vi "PicoScope3000aExampleRapidBlockBulkOverlapped.vi"() -> ()   [LabVIEW 2010]
uses:
  shared/PicoBuffers.ctl
  <vilib>/Waveform/DWDTOps.llb/DWDT Analog to Digital.vi
  shared/Segment Range.ctl
  shared/Buffer and Transfer Settings.ctl
  shared/Acquisition Settings.ctl
  shared/nSegments.ctl
  PicoScope3000aLib/PicoScope3000aDigitalChannelSettings.ctl
  PicoScope3000aLib/PicoScope3000aAnalogChannelSettings.ctl
panel:
  in  "Trigger Settings":T1={"Trigger Enabled"=FALSE, "Trigger Source"=enum."Channel A", "Trigger Threshold (volts)"=0.0, "Trigger Direction"=2, "Trigger Delay (samples)"=0, "Auto Trigger Time (ms)"=1000} {"Trigger Direction" items=["Above", "Below", "Rising", "Falling", "Rising or Falling"]}
  in  "Channel A Settings":T2={"Enabled"=TRUE, "Coupling"=1, "Range"=6, "Analogue Offset"=0.0, "Bandwidth Limit"=0} {"Bandwidth Limit" items=["Full", "20MHz"]; "Range" items=["10 mV", "20 mV", "50 mV", "100 mV", "200 mV", "500 mV", "1 V", "2 V", "5 V", "10 V", "20 V", "50 V ", "100 V"]; "Coupling" items=["AC", "DC"]}
  out "overflow":i16[](array[numeric]) format="%06b"
  in  "Port 0 Settings":T3={"Enabled"=FALSE, "Logic Level"=9830} {"Logic Level" items=["1.5V TTL"=9830, "2.5V CMOS"=16383]}
  out "USB 3.0 device on non-USB 3.0 Port":bool
  out "USB Powered":bool=TRUE
  out "Device Info":T4={"Driver Version"="2.1.104.3324", "USB Version"="2.0", "Hardware"="1", "Variant"="5244A", "Batch and Serial"="CQ178/007", "Cal Date"="11Jun13", "Kernel Version"="1.0", "Digital HW Version"="1", "Analogue HW Version"="1", "MSO"=FALSE, "Number of channels"=2}
  in  "Stop Display":bool
  out "Capture Complete":bool
  in  "Run":bool
  in  "Display Buffer Index":i32
  in  "Segment Range":T5={"fromSegmentIndex"=0, "toSegmentIndex"=9} {"toSegmentIndex" format="%.4p"; "fromSegmentIndex" format="%.4p"}
  in  "nSegments":T6=10 format="%.4p"
  out "error out":errorcluster
  in  "Data file":path=path "PicoScope3000aExampleRapidBlock ChA Data"
  in  "Buffer and Transfer Settings":T7={"startIndex"=0, "Samples"=5000000, "Down Sample Ratio"=1, "Down-Sample Mode"=0} {"Down-Sample Mode" items=["RAW none"=2147483648, "None"=0, "Aggregate"=1, "Decimate"=2, "Average"=4]; "Down Sample Ratio" step=1; "Samples" format="%_6p"}
  in  "Acquisition Settings":T8={"preTriggerSamples"=0, "postTriggerSamples"=5000000, "timebase"=5} {"postTriggerSamples" format="%_6p"; "preTriggerSamples" format="%_6p"}
  out "Properties Panel":T9={"Sample Frequency"=41666668.0, "Sample Rate"=2.4000000209412065e-08, "Max Samples Available"=26843008, "Number of Samples"=0, "Total Capture Time (sec) "=0.0, "Max Total Capture Time Available (sec)"=0.6442322134971619} {"Max Total Capture Time Available (sec)" format="%.3p"; "Sample Frequency" format="%.6p"; "Sample Rate" format="%.3p"; "Max Samples Available" format="%_6p"; "Total Capture Time (sec)" format="%.3p"}
  out "Port 0":digitalwaveform(graph)={"t0"=timestamp(0 s since 1904-01-01), "dt"=8e-09, "Y"={"transitions"=[], "data"=[]}}
  in  "stop":bool
  out "Analog Channels":cluster{i32, sgl, "Data":dbl[]}[](graph)
  in  "Serial Number":string
  in  "Use Serial Number":bool
  in  "error in (no error)":errorcluster
  # "Number of\nSegments to Capture"
  # "Bit 0 = ChA"
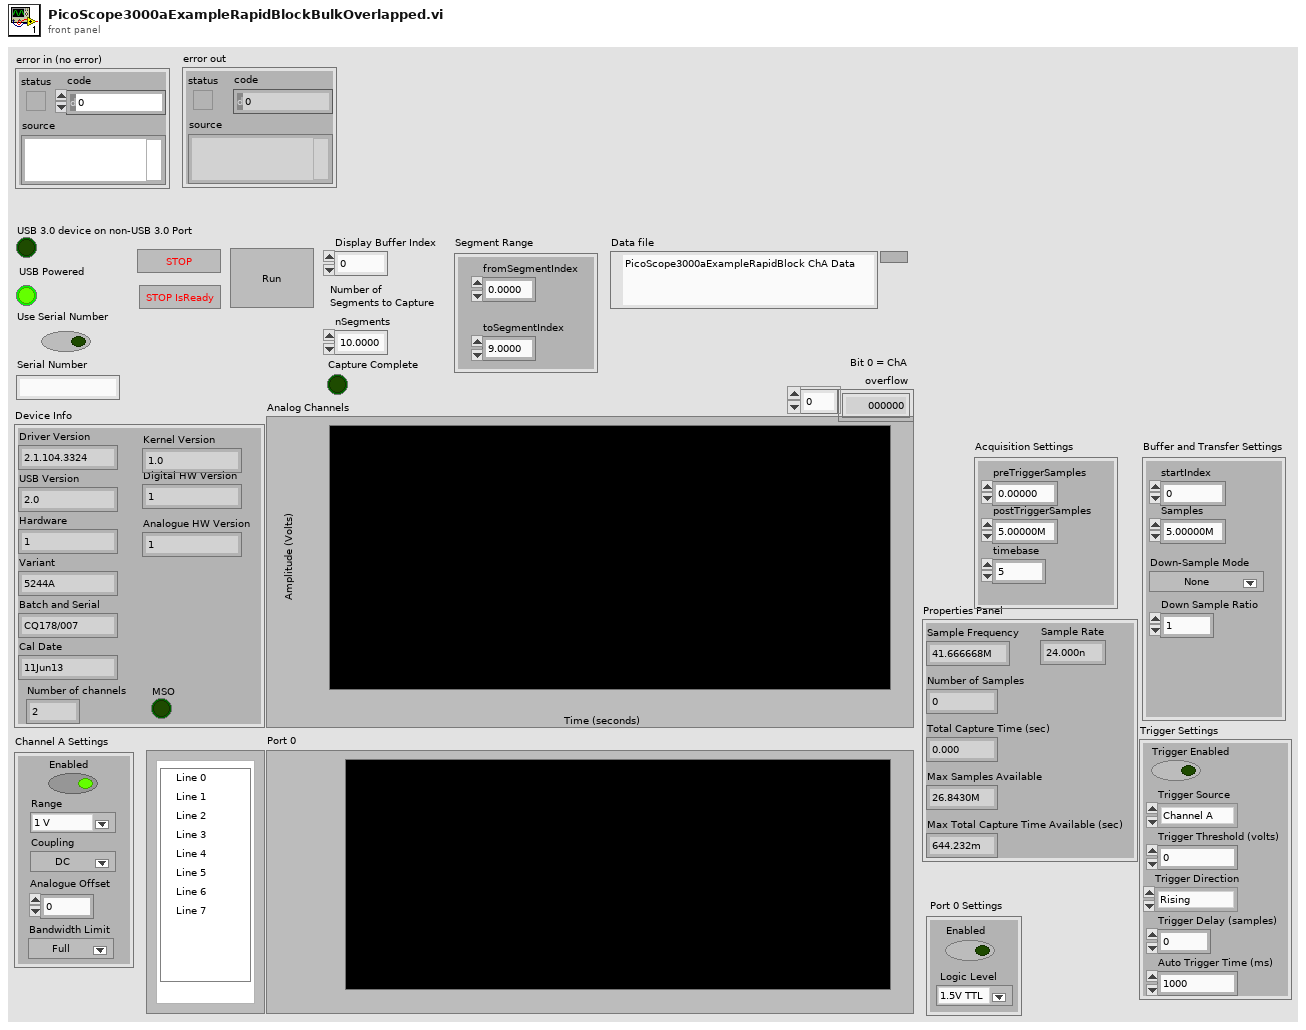
[diagram p1: front panel]
types:
  T1 = cluster{"Trigger Enabled":bool, "Trigger Source":enum32{"Channel A", "Channel B", "Channel C", "Channel D", "Ext."}, "Trigger Threshold (volts)":dbl, "Trigger Direction":u32, "Trigger Delay (samples)":u32, "Auto Trigger Time (ms)":i16}
  T2 = typedef "PicoScope3000aAnalogChannelSettings.ctl" = cluster{"Enabled":bool, "Coupling":u32, "Range":u32, "Analogue Offset":sgl, "Bandwidth Limit":u32}
  T3 = typedef "PicoScope3000aDigitalChannelSettings.ctl" = cluster{"Enabled":bool, "Logic Level":i16}
  T4 = cluster{"Driver Version":string, "USB Version":string, "Hardware":string, "Variant":string, "Batch and Serial":string, "Cal Date":string, "Kernel Version":string, "Digital HW Version":string, "Analogue HW Version":string, "MSO":bool, "Number of channels":i16}
  T5 = typedef "Segment Range.ctl" = cluster{"fromSegmentIndex":u64, "toSegmentIndex":u64}
  T6 = typedef "nSegments.ctl" = u64
  T7 = typedef "Buffer and Transfer Settings.ctl" = cluster{"startIndex":u64, "Samples":u64, "Down Sample Ratio":u64, "Down-Sample Mode":u32}
  T8 = typedef "Acquisition Settings.ctl" = cluster{"preTriggerSamples":u64, "postTriggerSamples":u64, "timebase":u32}
  T9 = cluster{"Sample Frequency":dbl, "Sample Rate":dbl, "Max Samples Available":u64, "Number of Samples":u64, "Total Capture Time (sec) ":dbl, "Max Total Capture Time Available (sec)":dbl}
  T10 = enum16{"open", "open or create", "create or replace", "create", "open (read-only)"}
  T11 = typedef "PicoBuffers.ctl" = cluster{"Max Buffer Pointers":u64[][][], "Min Buffer Pointers":u64[][][], "StreamingDataInfo":cluster{"Channel":u32, "Down-Sample Mode":u32, "PICO_DATA_TYPE":enum32{"PICO_INT8_T", "PICO_INT16_T", "PICO_INT32_T", "PICO_UINT32_T", "PICO_INT64_T", ""}, "Samples":i32, "bufferIndex":u64, "startIndex":i32, "overflow":i16}[][]}
  T12 = cluster{"Sample Frequency":sgl, "Sample Rate":sgl, "Max Samples Available":i32, "Number of Samples":u32, "Total Capture Time (sec) ":sgl, "Max Total Capture Time Available (sec)":sgl}
  T13 = cluster{"Channel A Buffer":i16[], "Channel B Buffer":i16[], "Channel C Buffer":i16[], "Channel D Buffer":i16[], "Channel E Buffer":i16[], "Channel F Buffer":i16[], "Channel G Buffer":i16[], "Channel H Buffer":i16[], "Port 0 Buffer":i16[], "Port 1 Buffer":i16[]}[]
  T14 = cluster{"Channel A Buffer":i16[], "Channel B Buffer":i16[], "Channel C Buffer":i16[], "Channel D Buffer":i16[], "Channel E Buffer":i16[], "Channel F Buffer":i16[], "Channel G Buffer":i16[], "Channel H Buffer":i16[], "Port 0 Buffer":i16[], "Port 1 Buffer":i16[]}
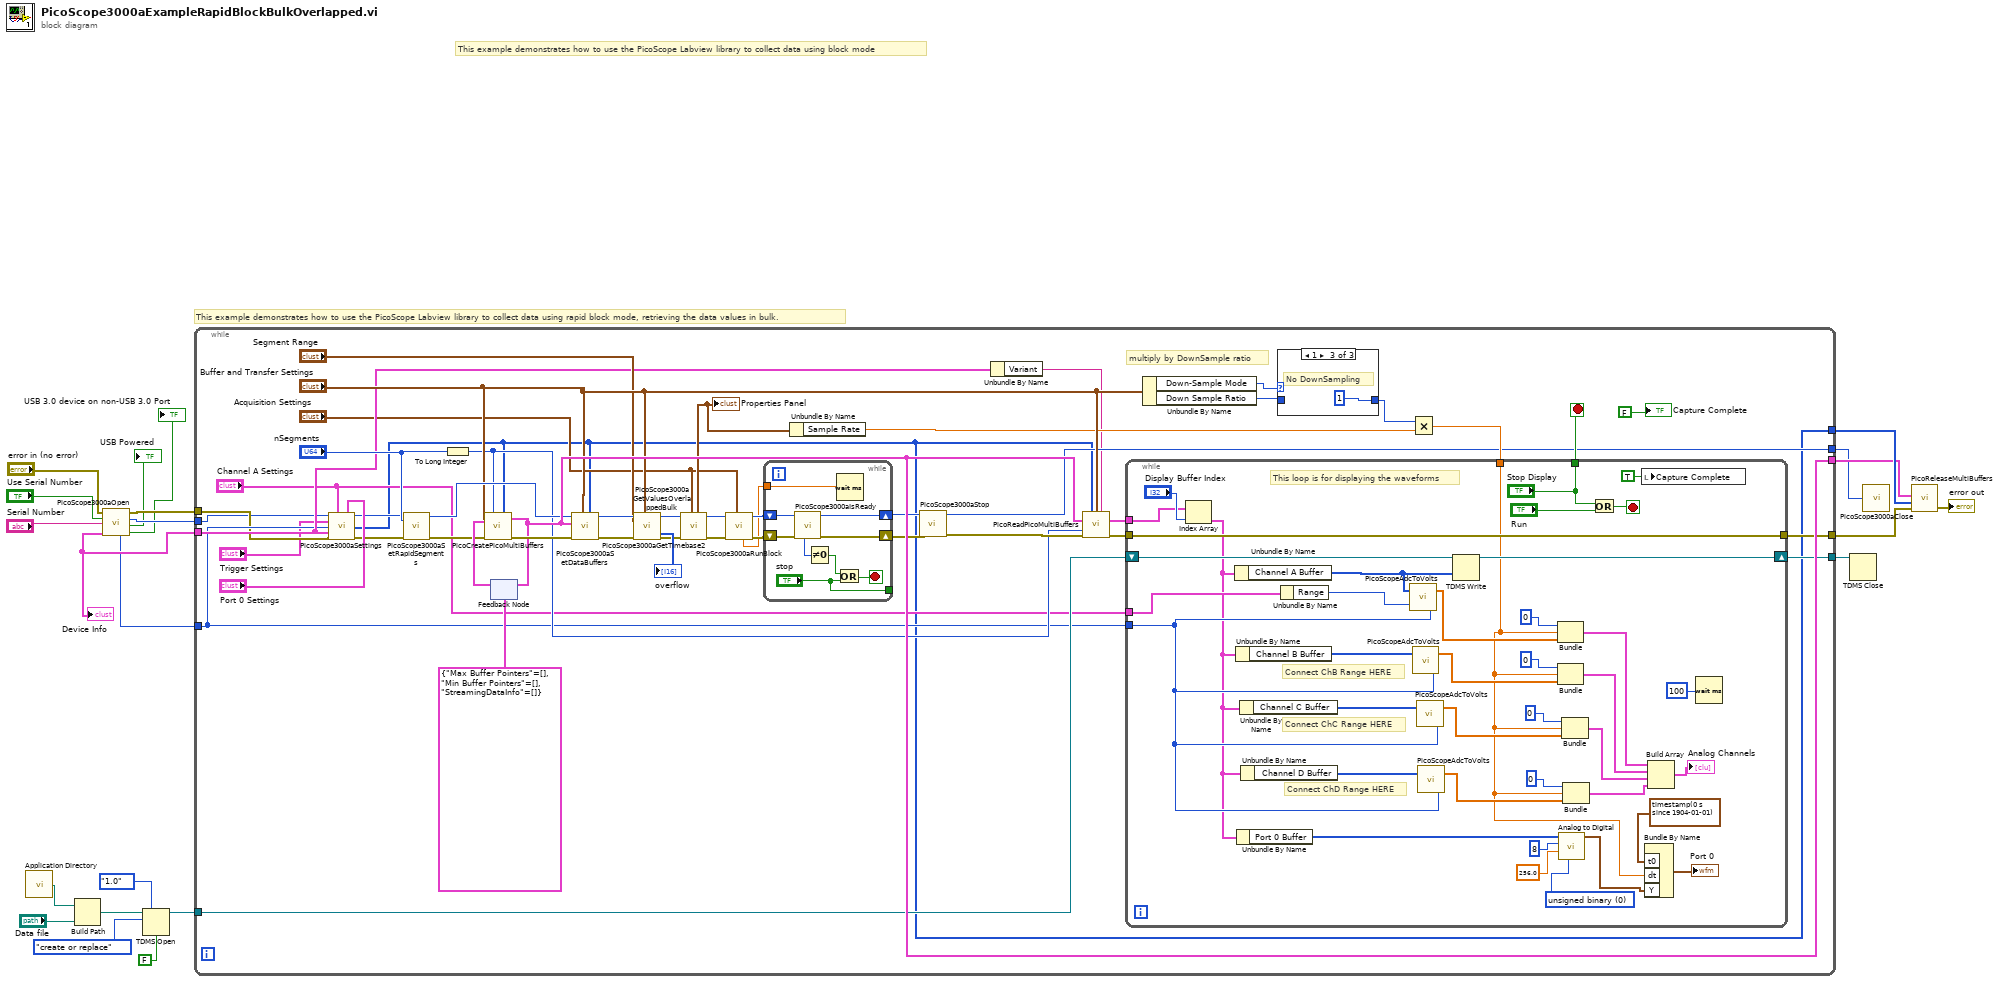
[diagram p0: block diagram]
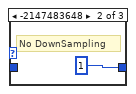
[diagram p3: hidden frame]
diagram:
  # "This example demonstrates how to use the PicoScope Labview library to collect data using rapid block mode, retrieving the data values in bulk."
  # "This example demonstrates how to use the PicoScope Labview library to collect data using block mode"
  n1 = call <vilib>:"Application Directory.vi"() -> ("Application Directory"=w13:path)
  n2 = Build Path(base path=w13, name or relative path="Data file") -> (appended path=w14:path)
  n3 = call "PicoScope3000aOpen.vi"("Batch/Serial"="Serial Number", "Use Serial number"="Use Serial Number", "error in (no error)"="error in (no error)") -> ("USB 3.0 device on non-USB 3.0 Port"=→"USB 3.0 device on non-USB 3.0 Port":bool, "USB Powered"=→"USB Powered":bool, "handle"=w22:i16, "error out"=w5:errorcluster, "Max ADC value"=w3:i16, "Device Info"=w6:T4)  [unwired: 3 in]
  "Device Info" <- w6
  n4 = TDMS Open(6:FALSE ("disable buffering? (T)"), 7:enum16{"1.0", "2.0"}."1.0" ("file format version (2.0)"), 10:T10."create or replace" ("operation (0:open)"), 11:w14) -> (3:w11:refnum<k34>)  [unwired: 2 in, 1 out]
  n5 = while {
    tunnel: w22 -> [w27]
    tunnel: w3 -> [w36]
    tunnel: [w46] -> w19
    tunnel: [w23] -> w21
    tunnel: [w68] -> w20
    tunnel: [w67] -> w12
    tunnel: w11 -> [w66]
    tunnel: w6 -> [w38]
    tunnel: w5 -> [w28]
    tunnel: [w44] -> w4
    stop <- w51 stop-if-true
    # "multiply by DownSample ratio"
    n6 = call "PicoScope3000aSettings.vi"("handle in"=w27, "Channel A Settings"="Channel A Settings", "Port 0 Settings"="Port 0 Settings", "Trigger Settings"="Trigger Settings", "Max_adc"=w36, "Device Info"=w38, "error in"=w28) -> ("handle out"=w25:i16, "Enabled Array"=w23:i16[], "error out"=w24:errorcluster)  [unwired: 6 in]
    n7 = call "PicoScope3000aSetRapidSegments.vi"("nSegments"="nSegments", "error in (no error)"=w24, "handle in"=w25) -> ("error out"=w65:errorcluster, "handle out"=w64:i16)  [unwired: 6 in, 1 out]
    n8 = To Long Integer(number="nSegments") -> (32bit integer=w43:i32)
    n9 = feedback #1(T11 {"Max Buffer Pointers"=[], "Min Buffer Pointers"=[], "StreamingDataInfo"=[]} ("Data Pointers")) -> (w70:T11)
    n10 = call "PicoCreatePicoMultiBuffers.vi"("Number of Buffers"=w43, "Buffer and Transfer Settings"="Buffer and Transfer Settings", "enabled array"=w23, "Data Pointers In"=w70, "error in (no error)"=w65) -> ("Data Pointers"=w68:T11, "error out"=w69:errorcluster)  [unwired: 9 in]
    n11 = feedback-in #1(w68) -> ()
    n12 = call "PicoScope3000aSetDataBuffers.vi"("enabled array"=w23, "Buffer and Transfer Settings"="Buffer and Transfer Settings", "error in (no error)"=w69, "Data Pointers In"=w68, "handle in"=w64) -> ("error out"=w63:errorcluster, "handle out"=w62:i16)  [unwired: 5 in]
    n13 = call "PicoScope3000aGetValuesOverlappedBulk.vi"("Segment Range"="Segment Range", "Buffer and Transfer Settings"="Buffer and Transfer Settings", "error in (no error)"=w63, "handle in"=w62) -> ("error out"=w32:errorcluster, "handle out"=w31:i16, "overflow"=→"overflow":i16[])  [unwired: 4 in, 1 out]
    n14 = call "PicoScope3000aGetTimebase2.vi"("Acquisition Settings"="Acquisition Settings", "error in (no error)"=w32, "handle in"=w31) -> ("error out"=w29:errorcluster, "handle out"=w30:i16, "Properties Panel"=w57:T12)  [unwired: 6 in]
    "Properties Panel" <- w57
    n15 = call "PicoScope3000aRunBlock.vi"("Acquisition Settings"="Acquisition Settings", "error in (no error)"=w29, "handle in"=w30) -> ("error out"=w54:errorcluster, "handle out"=w53:i16, "timeIndisposedMs"=w37:dbl)  [unwired: 5 in, 1 out]
    n16 = while {
      shift-right: [w118] -> w48
      shift-left: w54 -> [w119]
      shift-right: [w117] -> w45
      shift-left: w53 -> [w116]
      tunnel: ["stop"] -> _
      tunnel: w37 -> [w111]
      stop <- w113 stop-if-true
      n17 = call "PicoScope3000aIsReady.vi"("error in (no error)"=w119, "handle in"=w116) -> ("error out"=w118:errorcluster, "handle out"=w117:i16, "ready"=w115:i16)  [unwired: 7 in]
      n18 = Not Equal To 0?(x=w115) -> (x != 0?=w114:bool)
      n19 = Wait (ms)(milliseconds to wait=w111) -> ()  [unwired: 1 out]
      n20 = Or(x=w114, y="stop") -> (x .or. y?=w113:bool)
    }
    n21 = Unbundle By Name(w57) -> ("Sample Rate"=w40:sgl)
    n22 = call "PicoScope3000aStop.vi"("error in (no error)"=w48, "handle in"=w45) -> ("error out"=w47:errorcluster, "handle out"=w46:i16)  [unwired: 8 in]
    n23 = Unbundle By Name(w38) -> ("Variant"=w39:string)
    n24 = call "PicoReadPicoMultiBuffers.vi"("enabled array"=w23, "Buffer and Transfer Settings"="Buffer and Transfer Settings", "Variant"=w39, "Data Pointers"=w68, "No of Buffers"=w43, "error in (no error)"=w47) -> ("MultiBuffers (Max or non-aggregated)"=w60:T13, "error out"=w52:errorcluster)  [unwired: 7 in, 1 out]
    n25 = Unbundle By Name("Buffer and Transfer Settings") -> ("Down-Sample Mode"=w58:u32, "Down Sample Ratio"=w59:u64)
    n26 = case shown="1" w58 {
      tunnel: [w120 u64 1 ("Down Sample Ratio") u64 1 ("Down Sample Ratio")] -> w55
      tunnel: w59 -> [w120 _ _]
      frame Default {
      }
      frame -2147483648 {
        # "No DownSampling"
      }
      frame 1 {
        # "No DownSampling"
      }
    }
    n27 = Multiply(x=w55, y=w40) -> (x*y=w56:sgl)
    n28 = while {
      tunnel: w36 -> [w73]
      tunnel: "Channel A Settings" -> [w110]
      tunnel: w60 -> [w83]
      tunnel: w56 -> [w75]
      shift-right: [w109] -> w67
      shift-left: w66 -> [w108]
      tunnel: [w89] -> w44
      tunnel: w52 -> [w89]
      tunnel: ["Stop Display"] -> w51
      stop <- w86 stop-if-true
      w98 = u16 0 items=["unsigned binary", "offset binary", "2's complement"] ("data format (offset binary)")
      # "This loop is for displaying the waveforms"
      # "Connect ChB Range HERE"
      # "Connect ChD Range HERE"
      # "Connect ChC Range HERE"
      n29 = Index Array(array=w83, index="Display Buffer Index") -> (element=w72:T14)
      n30 = Unbundle By Name(w72) -> ("Channel A Buffer"=w91:i16[])
      n31 = Unbundle By Name(w72) -> ("Channel B Buffer"=w104:i16[])
      n32 = Unbundle By Name(w72) -> ("Port 0 Buffer"=w96:i16[])
      n33 = Unbundle By Name(w72) -> ("Channel C Buffer"=w81:i16[])
      n34 = Unbundle By Name(w72) -> ("Channel D Buffer"=w77:i16[])
      n35 = Unbundle By Name(w110) -> ("Range"=w106:u32)
      n36 = call "PicoScopeAdcToVolts.vi"("Max_adc"=w73, "Range Index"=w106, "Data"=w91) -> ("Data"=w92:dbl[])
      n37 = call "PicoScopeAdcToVolts.vi"("Max_adc"=w73, "Data"=w104) -> ("Data"=w103:dbl[])  [unwired: 1 in]
      n38 = call "PicoScopeAdcToVolts.vi"("Max_adc"=w73, "Data"=w81) -> ("Data"=w80:dbl[])  [unwired: 1 in]
      n39 = call "PicoScopeAdcToVolts.vi"("Max_adc"=w73, "Data"=w77) -> ("Data"=w76:dbl[])  [unwired: 1 in]
      n40 = TDMS Write(0:w108, 9:w91) -> (4:w109:refnum<k34>)  [unwired: 4 in, 3 out]
      n41 = Bundle(0, w75, "Data"=w92) -> (w102:cluster{i32, sgl, "Data":dbl[]})  [unwired: 1 in]
      n42 = Bundle(0, w75, "Data"=w103) -> (w101:cluster{i32, sgl, "Data":dbl[]})  [unwired: 1 in]
      n43 = call-poly <vilib>:"Analog to Digital.vi"("data format (offset binary)"=w98, "full-scale range (pk-pk)"=256.0, "resolution (16 bit)"=8, "analog waveform"=w96) -> ("digital waveform"=w93:digitalwaveform)  [unwired: 4 in, 3 out]
      n44 = Bundle(0, w75, "Data"=w80) -> (w79:cluster{i32, sgl, "Data":dbl[]})  [unwired: 1 in]
      n45 = Bundle(0, w75, "Data"=w76) -> (w74:cluster{i32, sgl, "Data":dbl[]})  [unwired: 1 in]
      n46 = Or(x="Stop Display", y="Run") -> (x .or. y?=w86:bool)
      n47 = local write "Capture Complete"(TRUE ("Capture Complete")) -> ()
      n48 = Bundle By Name("t0"=timestamp(0 s since 1904-01-01), "dt"=w75, "Y"=w93) -> (→"Port 0":digitalwaveform)  [unwired: 1 in]
      n49 = Build Array(w102, w101, w79, w74) -> (→"Analog Channels":cluster{i32, sgl, "Data":dbl[]}[])
      n50 = Wait (ms)(milliseconds to wait=u32 100) -> ()  [unwired: 1 out]
    }
    "Capture Complete" <- FALSE ("Capture Complete")
  }
  n51 = TDMS Close(11:w12) -> ()  [unwired: 1 in, 2 out]
  n52 = call "PicoScope3000aClose.vi"("handle"=w19) -> ()
  n53 = call "PicoReleaseMultiBuffers.vi"("error in (no error)"=w4, "Enabled array"=w21, "Data Pointers"=w20) -> ("error out"=→"error out":errorcluster)  [unwired: 8 in]
